vi "UnscentedKalmanFilter_New_FuncGroup.vi"(0 "addFuncXExtra":variant, 3 "MeanFuncX":T2, 4 "AddFuncX":T2, 5 "MeanFuncXExtra":variant, 6 "residualFuncYExtra":variant, 7 "MeanFuncY":T2, 8 "ResidualFuncY":T2, 9 "residualFuncXExtra":variant, 10 "ResidualFuncX":T2, 11 "MeanFuncYExtra":variant) -> (1 "Error":errorcluster, 2 "UNSCENTED_KALMAN_NEW_FUNC_GROUP":T1)   [LabVIEW 2019, in "Trajectory_Library.lvlib"]
doc: "Creates a new packed function group cluster .\n \nInputs:\n - meanFuncX -- A strict function reference that computes the mean of 2States + 1 state vectors using a given set of weights.\n - meanFuncXExtra -- A variant containing extra data for the meanX function\n - meanFuncY -- A strict function reference that computes the mean of 2 States + 1 measurement vectors using a given set of weights.\n - meanFuncYExtra -- A variant containing extra data for the meanY function\n - residualFuncX -- A strict function reference that computes the residual of two state vectors (i.e. it subtracts them.)\n - residualFuncXExtra -- A variant containing extra data for the residualX function\n - residualFuncY -- A strict function reference that computes the residual of two measurement vectors (i.e. it subtracts them.)\n - residualFuncYExtra -- A variant containing extra data for the residualY function\n - addFuncX -- A strict function reference that adds two state vectors.\n - addFuncXExtra -- A variant containing extra data for the addX function\n\nOutputs:\n - UnscentedKalmanFilterFuncGroup -- Cluster containing the functions and extra data.\n - Error -- If TRUE, an error occured."
uses:
  Trajectory_Library.lvlib
  TypeDef/CALLBACK_FUNC_TYPE.ctl
  TypeDef/UNSCENTED_KALMAN_NEW_FUNC_GROUP.ctl
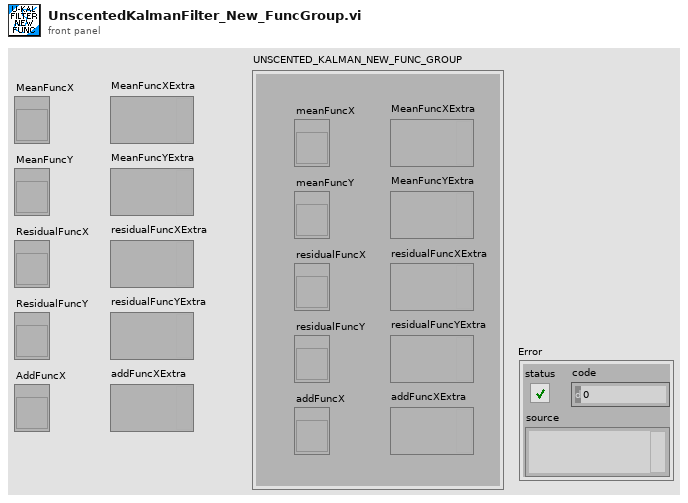
[diagram p1: front panel]
types:
  T1 = typedef "Trajectory_Library.lvlib/UNSCENTED_KALMAN_NEW_FUNC_GROUP.ctl" = cluster{"meanFuncX":T2, "meanFuncY":T2, "residualFuncX":T2, "residualFuncY":T2, "addFuncX":T2, "MeanFuncXExtra":variant, "MeanFuncYExtra":variant, "residualFuncXExtra":variant, "residualFuncYExtra":variant, "addFuncXExtra":variant}
  T2 = typedef "Trajectory_Library.lvlib/CALLBACK_FUNC_TYPE.ctl" = refnum<vi>
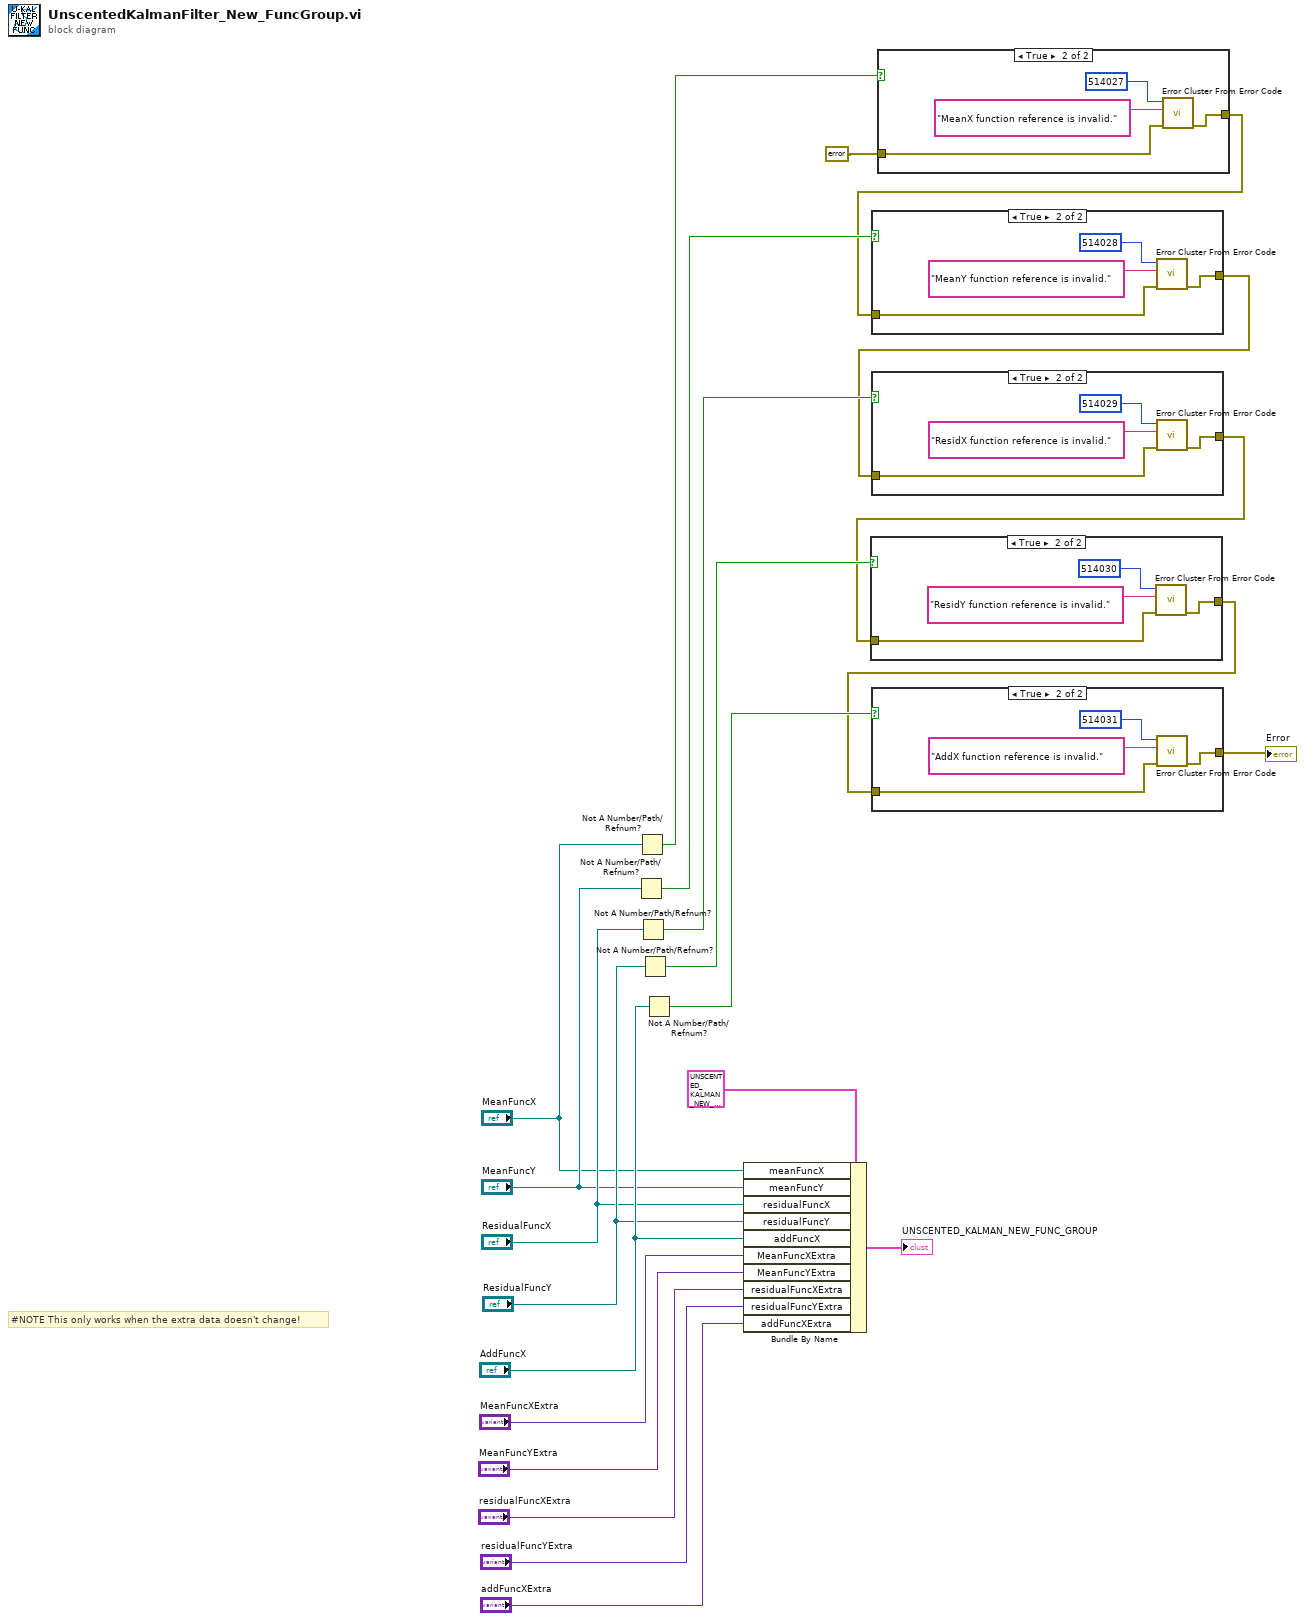
[diagram p0: block diagram]
diagram:
  # "#NOTE This only works when the extra data doesn't change!"
  n1 = Not A Number/Path/Refnum?(number/path/refnum="MeanFuncY") -> (NaN/Path/Refnum?=w9:bool)
  n2 = Not A Number/Path/Refnum?(number/path/refnum="MeanFuncX") -> (NaN/Path/Refnum?=w10:bool)
  n3 = Not A Number/Path/Refnum?(number/path/refnum="ResidualFuncX") -> (NaN/Path/Refnum?=w8:bool)
  n4 = Not A Number/Path/Refnum?(number/path/refnum="ResidualFuncY") -> (NaN/Path/Refnum?=w7:bool)
  n5 = Not A Number/Path/Refnum?(number/path/refnum="AddFuncX") -> (NaN/Path/Refnum?=w6:bool)
  n6 = Bundle By Name(cluster=T1 {"meanFuncX"=refnum, "meanFuncY"=refnum, "residualFuncX"=refnum, "residualFuncY"=refnum, "addFuncX"=refnum, "MeanFuncXExtra"=variant, "MeanFuncYExtra"=variant, "residualFuncXExtra"=variant, "residualFuncYExtra"=variant, "addFuncXExtra"=variant} ("UNSCENTED_KALMAN_FILTER_FUNC_GROUP"), "meanFuncX"="MeanFuncX", "meanFuncY"="MeanFuncY", "residualFuncX"="ResidualFuncX", "residualFuncY"="ResidualFuncY", "addFuncX"="AddFuncX", "MeanFuncXExtra"="MeanFuncXExtra", "MeanFuncYExtra"="MeanFuncYExtra", "residualFuncXExtra"="residualFuncXExtra", "residualFuncYExtra"="residualFuncYExtra", "addFuncXExtra"="addFuncXExtra") -> (→"UNSCENTED_KALMAN_NEW_FUNC_GROUP":T1)
  n7 = case shown="True" w10 {
    tunnel: errorcluster {"status"=FALSE, "code"=0, "source"=""} ("error constant") -> [w24 w27]
    tunnel: [w24 w28] -> w5
    frame False {
    }
    frame True {
      n8 = call <vilib>:"Error Cluster From Error Code.vi"("error in (no error)"=w27, "error message (\"\")"="MeanX function reference is invalid." ("error message (\"\")"), "error code (0)"=514027) -> ("error out"=w28:errorcluster)  [unwired: 6 in]
    }
  }
  n9 = case shown="True" w9 {
    tunnel: w5 -> [w29 w32]
    tunnel: [w29 w33] -> w4
    frame False {
    }
    frame True {
      n10 = call <vilib>:"Error Cluster From Error Code.vi"("error in (no error)"=w32, "error message (\"\")"="MeanY function reference is invalid." ("error message (\"\")"), "error code (0)"=514028) -> ("error out"=w33:errorcluster)  [unwired: 6 in]
    }
  }
  n11 = case shown="True" w8 {
    tunnel: w4 -> [w34 w37]
    tunnel: [w34 w38] -> w3
    frame False {
    }
    frame True {
      n12 = call <vilib>:"Error Cluster From Error Code.vi"("error in (no error)"=w37, "error message (\"\")"="ResidX function reference is invalid." ("error message (\"\")"), "error code (0)"=514029) -> ("error out"=w38:errorcluster)  [unwired: 6 in]
    }
  }
  n13 = case shown="True" w7 {
    tunnel: w3 -> [w39 w42]
    tunnel: [w39 w43] -> w2
    frame False {
    }
    frame True {
      n14 = call <vilib>:"Error Cluster From Error Code.vi"("error in (no error)"=w42, "error message (\"\")"="ResidY function reference is invalid." ("error message (\"\")"), "error code (0)"=514030) -> ("error out"=w43:errorcluster)  [unwired: 6 in]
    }
  }
  n15 = case shown="True" w6 {
    tunnel: w2 -> [w44 w47]
    tunnel: [w44 w48] -> w1
    frame False {
    }
    frame True {
      n16 = call <vilib>:"Error Cluster From Error Code.vi"("error in (no error)"=w47, "error message (\"\")"="AddX function reference is invalid." ("error message (\"\")"), "error code (0)"=514031) -> ("error out"=w48:errorcluster)  [unwired: 6 in]
    }
  }
  "Error" <- w1
